vi "RemoteVI Complex Fixture Paste.vi"(0 "Fixture":path, 1 "Donors":path[](array[path]), 2 "Donor Labels":string[](array[string]), 3 "Labels":string[](array[string]), 5 "Pane":i32[](array[numeric]), 11 "error in":errorcluster) -> (15 "error out":errorcluster)   [LabVIEW 2020]
doc: "Build tool of RemoteVI Complex Fixture.vi: run it ONCE after the graft (see compose_complex.py), with the fixture idle. AIXML cannot create a tab control, a subpanel, a slide, a knob, a tree or a graph with cursors (the composer's slide and knob parts crash LabVIEW 2025 on load), so this copies them from other VIs onto the fixture's panel, into the pane given by Pane (0 left, 1 toolbar, 2 main, the order of Panes[] on NI's splitter example) at Position, and relabels them: for each row of Donors, the control labelled Donor Labels is selected on the donor's panel, copied (Copy Selection) and pasted (Paste Selection with the pane), then found on the fixture by its donor label and given its new label. Saves the fixture. Run Arrange afterwards."
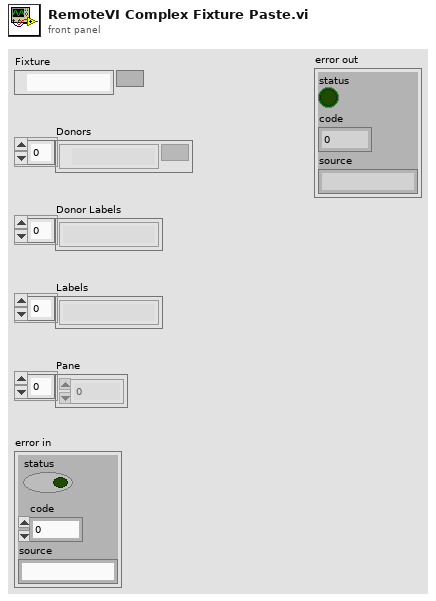
[diagram p1: front panel]
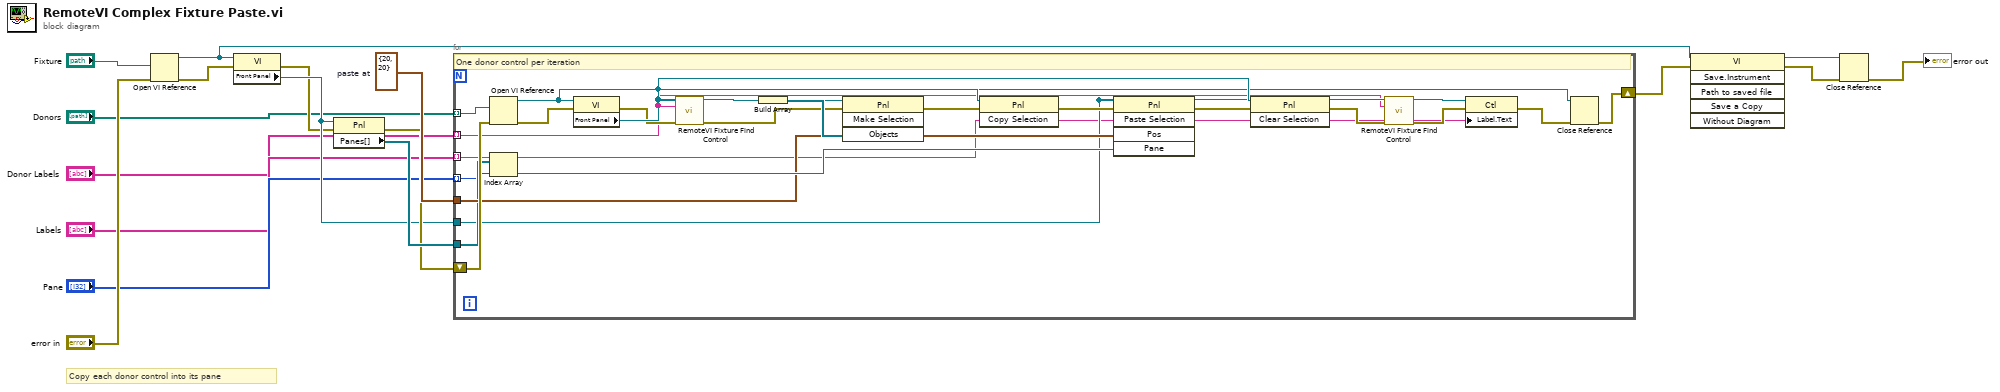
[diagram p0: block diagram]
diagram:
  w13 = cluster{"Left":i32, "Top":i32} {"Left"=20, "Top"=20}  # paste at
  # "Copy each donor control into its pane"
  n1 = Open VI Reference(vi path="Fixture", error in (no error)="error in") -> (vi reference=w7:refnum<vi>, error out=w8:errorcluster)  [unwired: 4 in]
  n2 = property class="VI"(reference=w7, error in=w8) -> (error out=w9:errorcluster, "Front Panel"=w10:refnum<vi>)  [unwired: 1 out]
  n3 = property class="Pnl"(reference=w10, error in=w9) -> (error out=w11:errorcluster, "Panes[]"=w12:refnum<vi>[])  [unwired: 1 out]
  n4 = for {
    tunnel: "Donors" -> [w18] mode=indexing
    tunnel: "Donor Labels" -> [w19] mode=indexing
    tunnel: "Labels" -> [w20] mode=indexing
    tunnel: "Pane" -> [w21] mode=indexing
    tunnel: w13 -> [w24]
    tunnel: w10 -> [w22]
    tunnel: w12 -> [w23]
    shift-right: [w26] -> w14
    shift-left: w11 -> [w25]
    # "One donor control per iteration"
    n5 = Open VI Reference(vi path=w18, error in (no error)=w25) -> (vi reference=w27:refnum<vi>, error out=w28:errorcluster)  [unwired: 4 in]
    n6 = Index Array(array=w23, index=w21) -> (element=w36:refnum<vi>)
    n7 = property class="VI"(reference=w27, error in=w28) -> (error out=w29:errorcluster, "Front Panel"=w30:refnum<vi>)  [unwired: 1 out]
    n8 = call "RemoteVI Fixture Find Control.vi"("Panel"=w30, "label"=w19, "error in"=w29) -> ("Control Ref"=w31:refnum<vi>, "error out"=w32:errorcluster)  [unwired: 11 in]
    n9 = Build Array(w31) -> (w33:refnum<vi>[])
    n10 = invoke class="Pnl" method="Make Selection"(reference=w30, error in=w32, "Objects"=w33) -> (error out=w34:errorcluster)  [unwired: 1 in, 3 out]
    n11 = invoke class="Pnl" method="Copy Selection"(reference=w30, error in=w34) -> (error out=w35:errorcluster)  [unwired: 1 in, 2 out]
    n12 = invoke class="Pnl" method="Paste Selection"(reference=w22, error in=w35, "Pos"=w24, "Pane"=w36) -> (error out=w37:errorcluster)  [unwired: 1 in, 4 out]
    n13 = invoke class="Pnl" method="Clear Selection"(reference=w30, error in=w37) -> (error out=w38:errorcluster)  [unwired: 1 in, 2 out]
    n14 = call "RemoteVI Fixture Find Control.vi"("Panel"=w22, "label"=w19, "error in"=w38) -> ("Control Ref"=w39:refnum<vi>, "error out"=w40:errorcluster)  [unwired: 11 in]
    n15 = property class="Ctl"(reference=w39, error in=w40, "Label.Text"=w20) -> (error out=w41:errorcluster)  [unwired: 1 out]
    n16 = Close Reference(reference=w27, error in (no error)=w41) -> (error out=w26:errorcluster)
  }
  n17 = invoke class="VI" method="Save.Instrument"(reference=w7, error in=w14) -> (reference out=w15:refnum<vi>, error out=w16:errorcluster)  [unwired: 4 in, 4 out]
  n18 = Close Reference(reference=w15, error in (no error)=w16) -> (error out=→"error out":errorcluster)
